vi "MQTT Client - Publish.vi"(0 "MQTT Session":T3, 1 "Retain":bool, 5 "Topic":string, 7 "Message":string, 9 "QoS":T2, 11 "error in":errorcluster, 12 "Publish Properties (v5)":T1[](array[typedef]) {"Property" items=[" Payload Format Indicator          "=1, " Message Expiry Interval           "=2, " Content Type                      "=3, " Response Topic                    "=8, " Correlation Data                  "=9, " Subscription Identifier           "=11, " Topic Alias                       "=35, " User Property                     "=38]}) -> (4 "MQTT Session out":T3, 15 "error out":errorcluster)   [LabVIEW 2019, in "KoRE-MQTT.lvlib"]
doc: "<b>Description:</b> This VI publishes messages to an MQTT broker. It takes various parameters such as topic, message content, and QoS level for sending the message.\n\n<b>Input Terminals:</b>\n- <b>Retain [1]</b>: Boolean value that specifies whether the message should be retained by the broker for future subscribers.\n- <b>MQTT Session [0]</b>: Reference to the established MQTT session for message publication.\n- <b>Topic [5]</b>: The specific topic to which the message will be published.\n- <b>Message [7]</b>: The actual message content that will be sent to the specified topic.\n- <b>QoS [9]</b>: Quality of Service level for message delivery, indicating the assurance of message delivery.\n- <b>Publish Properties (v5) [12]</b>: An array of Property and Value pairs specific to MQTT v5 connections that can be used for advanced message publication settings.\n\n<b>Output Terminals:</b>\n- <b>MQTT Session out [4]</b>: Reference to the MQTT session from which messages are to be published.\n\nCopyright (c) 2025 KoRElibs.com\nSPDX-License-Identifier: EUPL-1.2\n\nThis VI is licensed under the European Union Public License (EUPL) Version 1.2. You may use this VI unmodified in proprietary works. If you distribute a modified version of this file, the modified file must be released under the EUPL-1.2. Full license: https://joinup.ec.europa.eu/asset/eupl/eupl/1.2/"
uses:
  KoRE-MQTT.lvlib
  TypeDefs/MQTT Client Session.ctl
  TypeDefs/MQTT QoS Level.ctl
  TypeDefs/MQTT Property - PUBLISH.ctl
  Private/TypeDefs/MQTT Packet - Type.ctl
  Private/MQTT Session - Reset Keep Alive Timer.vi
  Private/MQTT Data Stream - Write Packet.vi
  Private/MQTT Data - Encode Varint.vi
panel:
  out "DEBUG":string
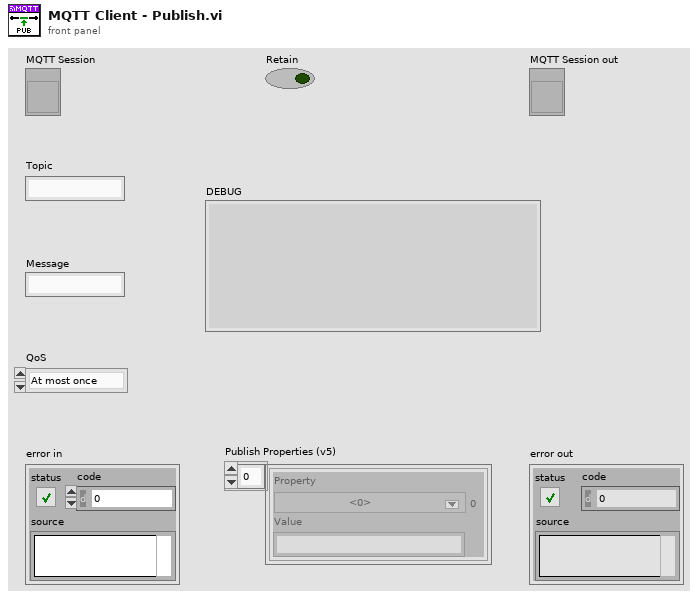
[diagram p1: front panel]
types:
  T1 = typedef "KoRE-MQTT.lvlib/MQTT Property - PUBLISH.ctl" = cluster{"Property":u8, "Value":string}
  T2 = typedef "KoRE-MQTT.lvlib/MQTT QoS Level.ctl" = enum8{"At most once", "At least once", "Exactly once"}
  T3 = typedef "KoRE-MQTT.lvlib/MQTT Client Session.ctl" = refnum<vi>
  T4 = typedef "KoRE-MQTT.lvlib/MQTT Packet - Type.ctl" = enum32{"Reserved", "CONNECT", "CONNACK", "PUBLISH", "PUBACK", "PUBREC", "PUBREL", "PUBCOMP", "SUBSCRIBE", "SUBACK", "UNSUBSCRIBE", "UNSUBACK", "PINGREQ", "PINGRESP", "DISCONNECT", "AUTH"}
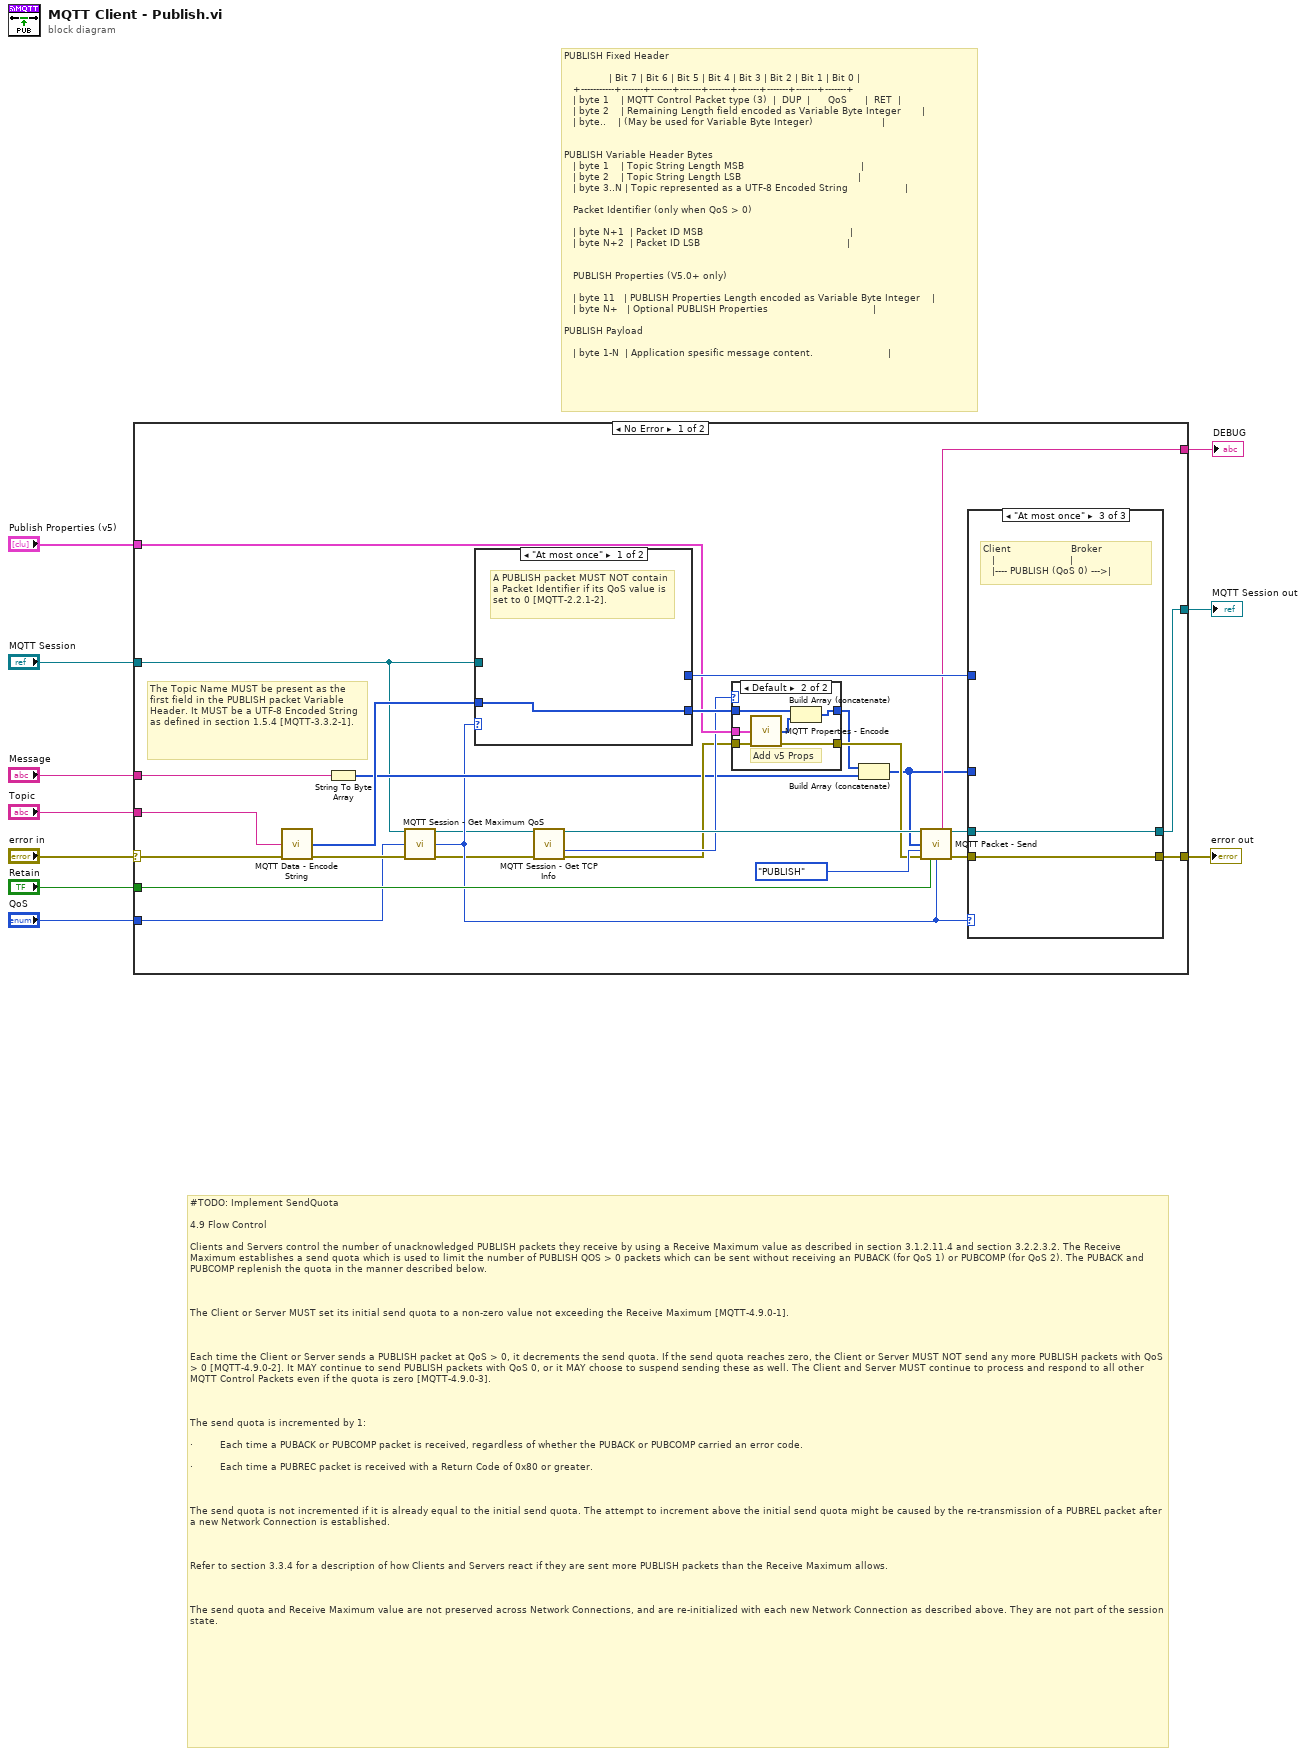
[diagram p0: block diagram]
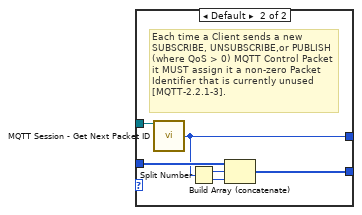
[diagram p2: hidden frame]
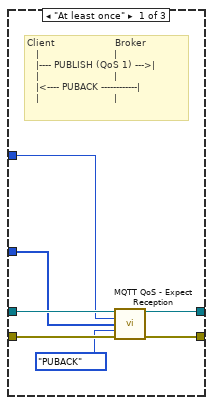
[diagram p4: hidden frame]
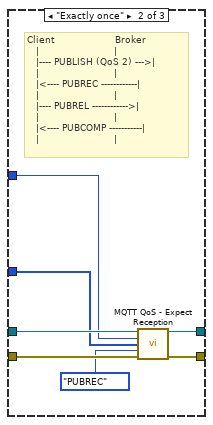
[diagram p5: hidden frame]
diagram:
  # "#TODO: Implement SendQuota\n\n4.9 Flow Control\n\nClients and Servers control the number of unacknowledged PUBLISH packets they receive by using a Receive Maximum value as described in section 3.1.2.11.4 and section 3.2.2.3.2. The Receive Maximum establishes a send quota which is used to limit the number of PUBLISH QOS > 0 packets which can be sent without receiving an PUBACK (for QoS 1) or PUBCOMP (for QoS 2). The PUBACK and PUBCOMP replenish the quota in the manner described below.\n\n \n\nThe Client or Server MUST set its initial send quota to a non-zero value not exceeding the Receive Maximum [MQTT-4.9.0-1].\n\n \n\nEach time the Client or Server sends a PUBLISH packet at QoS > 0, it decrements the send quota. If the send quota reaches zero, the Client or Server MUST NOT send any more PUBLISH packets with QoS > 0 [MQTT-4.9.0-2]. It MAY continue to send PUBLISH packets with QoS 0, or it MAY choose to suspend sending these as well. The Client and Server MUST continue to process and respond to all other MQTT Control Packets even if the quota is zero [MQTT-4.9.0-3].\n\n \n\nThe send quota is incremented by 1:\n\n·         Each time a PUBACK or PUBCOMP packet is received, regardless of whether the PUBACK or PUBCOMP carried an error code.\n\n·         Each time a PUBREC packet is received with a Return Code of 0x80 or greater.\n\n \n\nThe send quota is not incremented if it is already equal to the initial send quota. The attempt to increment above the initial send quota might be caused by the re-transmission of a PUBREL packet after a new Network Connection is established.\n\n \n\nRefer to section 3.3.4 for a description of how Clients and Servers react if they are sent more PUBLISH packets than the Receive Maximum allows.\n\n \n\nThe send quota and Receive Maximum value are not preserved across Network Connections, and are re-initialized with each new Network Connection as described above. They are not part of the session state."
  # "PUBLISH Fixed Header\n\n               | Bit 7 | Bit 6 | Bit 5 | Bit 4 | Bit 3 | Bit 2 | Bit 1 | Bit 0 |\n   +-----------+-------+-------+-------+-------+-------+-------+-------+-------+\n   | byte 1    | MQTT Control Packet type (3)  |  DUP  |      QoS      |  RET  |\n   | byte 2    | Remaining Length field encoded as Variable Byte Integer       |\n   | byte..    | (May be used for Variable Byte Integer)                       | \n\n\nPUBLISH Variable Header Bytes\n   | byte 1    | Topic String Length MSB                                       |  \n   | byte 2    | Topic String Length LSB                                       |  \n   | byte 3..N | Topic represented as a UTF-8 Encoded String                   |\n\n   Packet Identifier (only when QoS > 0)   \n\n   | byte N+1  | Packet ID MSB                                                 |  \n   | byte N+2  | Packet ID LSB                                                 |\n\n\n   PUBLISH Properties (V5.0+ only)\n\n   | byte 11   | PUBLISH Properties Length encoded as Variable Byte Integer    |\n   | byte N+   | Optional PUBLISH Properties                                   |\n\nPUBLISH Payload \n\n   | byte 1-N  | Application spesific message content.                         |"
  n1 = case shown="No Error" "error in" {
    selector: "error in" -> [w24 w70]
    tunnel: [w23 w70] -> w9
    tunnel: "MQTT Session" -> [w12 w69]
    tunnel: [w27 w69] -> w7
    tunnel: "Topic" -> [w37 _]
    tunnel: "Message" -> [w34 _]
    tunnel: "QoS" -> [w15 _]
    tunnel: "Retain" -> [w35 _]
    tunnel: "Publish Properties (v5)" -> [w31 _]
    tunnel: [w22 _] -> w1
    frame No Error {
      # "The Topic Name MUST be present as the first field in the PUBLISH packet Variable Header. It MUST be a UTF-8 Encoded String as defined in section 1.5.4 [MQTT-3.3.2-1]."
      n2 = call "MQTT Data - Encode String.vi"("String in"=w37, "error in (no error)"=w24) -> ("Bytes out"=w30:u8[], "error out"=w16:errorcluster)  [unwired: 12 in]
      n3 = String To Byte Array(string=w34) -> (unsigned byte array=w18:u8[])
      n4 = call "MQTT Session - Get Maximum QoS.vi"("MQTT Session"=w12, "QoS"=w15, "error in"=w16) -> ("MQTT Session Out"=w11:T3, "QoS"=w14:T2, "error out"=w13:errorcluster)  [unwired: 10 in]
      n5 = case shown="\"At most once\"" w14 {
        tunnel: w12 -> [_ w44]
        tunnel: w30 -> [w38 w41]
        tunnel: [w38 w40] -> w33
        tunnel: [_ w39] -> w32
        frame "At most once" {
          # "A PUBLISH packet MUST NOT contain a Packet Identifier if its QoS value is set to 0 [MQTT-2.2.1-2]."
        }
        frame Default {
          # "Each time a Client sends a new SUBSCRIBE, UNSUBSCRIBE,or PUBLISH (where QoS > 0) MQTT Control Packet it MUST assign it a non-zero Packet Identifier that is currently unused [MQTT-2.2.1-3]."
          n6 = call "MQTT Session - Get Next Packet ID.vi"("MQTT_Q In in"=w44) -> ("PacketID"=w39:u16)  [unwired: 13 in, 1 out]
          n7 = Split Number(x=w39) -> (hi(x)=w43:u8, lo(x)=w42:u8)
          n8 = Build Array (concatenate)(w41, w43, w42) -> (w40:u8[])
        }
      }
      n9 = call "MQTT Session - Get TCP Info.vi"("mqtt ref in"=w11, "error in"=w13) -> ("mqtt ref out"=w26:T3, "Version"=w25:u8, "error out"=w21:errorcluster)  [unwired: 9 in, 2 out]
      n10 = case shown="Default" w25 {
        tunnel: w33 -> [w46 w51]
        tunnel: [w46 w50] -> w19
        tunnel: w31 -> [_ w52]
        tunnel: w21 -> [w45 w48]
        tunnel: [w45 w47] -> w20
        frame 3, 4 {
        }
        frame Default {
          # "Add v5 Props"
          n11 = call "MQTT Properties - Encode.vi"("MQTT Properties"=w52, "error in (no error)"=w48) -> ("Encoded MQTT Properties"=w49:u8[], "error out"=w47:errorcluster)  [unwired: 12 in]
          n12 = Build Array (concatenate)(w51, w49) -> (w50:u8[])
        }
      }
      n13 = Build Array (concatenate)(w19, w18) -> (w17:u8[])
      n14 = call "MQTT Packet - Send.vi"("mqtt ref in"=w26, "packet data"=w17, "MessageType"=MQTT_Packet_-_Type."PUBLISH", "error in (no error)"=w20, "Retain"=w35, "QoS"=w14) -> ("Debug"=w22:string, "mqtt ref out"=w29:T3, "error out"=w28:errorcluster)  [unwired: 7 in]
      n15 = case shown="\"At most once\"" w14 {
        tunnel: [w56 w63 w68] -> w23
        tunnel: w28 -> [w58 w65 w68]
        tunnel: w32 -> [w55 w62 _]
        tunnel: w29 -> [w59 w66 w67]
        tunnel: [w57 w64 w67] -> w27
        tunnel: w17 -> [w53 w60 _]
        frame "At least once" {
          # "Client                    Broker\n   |                         |\n   |---- PUBLISH (QoS 1) --->|\n   |                         |\n   |<---- PUBACK ------------|\n   |                         |"
          n16 = call "MQTT QoS - Expect Reception.vi"("MQTT Reference"=w59, "Packet ID"=w55, "Message"=w53, "MessageType"=MQTT_Packet_-_Type."PUBACK", "Error In"=w58) -> ("MQTT Reference"=w57:T3, "Error Out"=w56:errorcluster)  [unwired: 8 in, 1 out]
        }
        frame "Exactly once" {
          # "Client                    Broker\n   |                         |\n   |---- PUBLISH (QoS 2) --->|\n   |                         |\n   |<---- PUBREC ------------|\n   |                         |\n   |---- PUBREL ------------>|\n   |                         |\n   |<---- PUBCOMP -----------|\n   |                         |"
          n17 = call "MQTT QoS - Expect Reception.vi"("MQTT Reference"=w66, "Packet ID"=w62, "Message"=w60, "MessageType"=MQTT_Packet_-_Type."PUBREC", "Error In"=w65) -> ("MQTT Reference"=w64:T3, "Error Out"=w63:errorcluster)  [unwired: 8 in, 1 out]
        }
        frame "At most once" {
          # "Client                    Broker\n   |                         |\n   |---- PUBLISH (QoS 0) --->|"
        }
      }
    }
    frame Error {
    }
  }
  "error out" <- w9
  "MQTT Session out" <- w7
  "DEBUG" <- w1
